vi "Drive Controller.vi"(8 "error in":errorcluster) -> ()   [LabVIEW 2023]
doc: "This VI executes continuously carrying out the current operation and responding to updates or new operation requests. It will often contain the timing or control code that is difficult to place directly in TeleOp. This VI generally opens all sensors and motors and isolates the rest of the robot code from knowing implementation details of how the operations are carried out."
uses:
  Drive Operations.ctl
  Drive Setpoints.ctl
  swerve-template/Type Definitions/Data/Robot Velocities.ctl
  Robot Global Data.vi
  80b923c8-6b82-42f9-a8cd-acddf0fa8107.vi
  Auto Data.ctl
  <vilib>/REV Custom Controls/Spark Output Control Type.ctl
  <vilib>/REVLibDriver/REVLibDriver.lvlib
panel:
  in  "Drive Controller Diagnostics":T1(tab)
  out "Swerve Visualizer":cluster{dbl[], dbl[]}[](graph)
  out "Pod Comparisons (Diff -> Setpoint - Actual)":T2
  out "(Calibration) Steering Angles":T3
  out "Current\nCmd":string
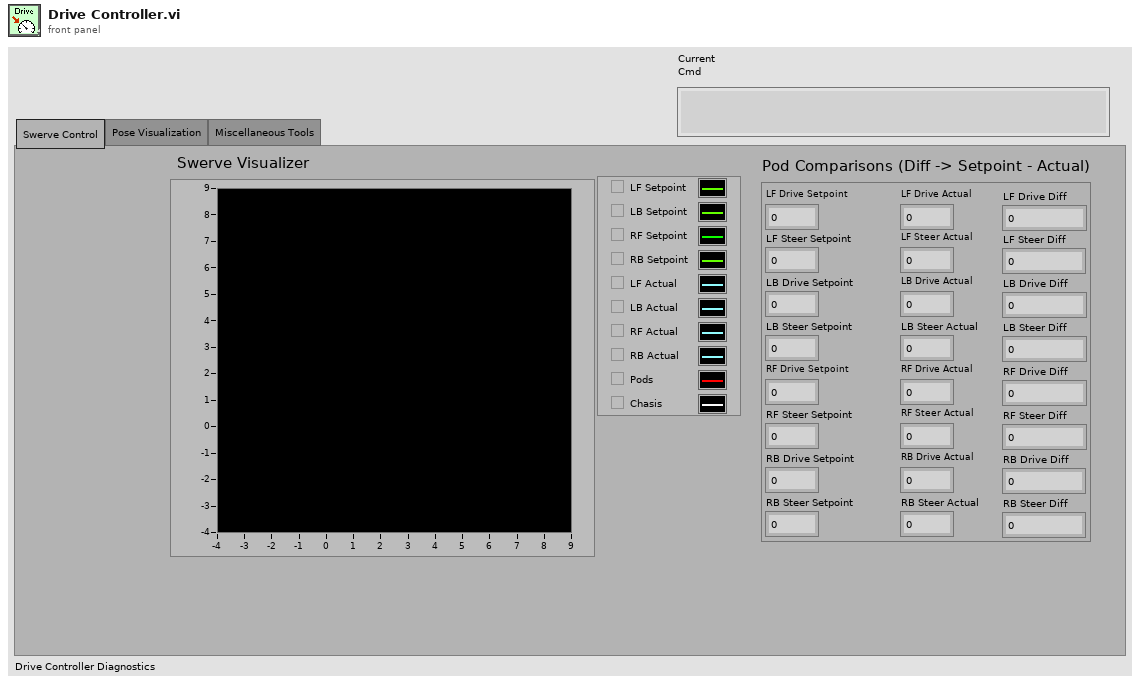
[diagram p1: front panel]
types:
  T1 = enum32{"Swerve Control", "Pose Visualization", "Miscellaneous Tools"}
  T2 = cluster{"LF Drive Setpoint":dbl, "LF Steer Setpoint":dbl, "LB Drive Setpoint":dbl, "LB Steer Setpoint":dbl, "RF Drive Setpoint":dbl, "RF Steer Setpoint":dbl, "RB Drive Setpoint":dbl, "RB Steer Setpoint":dbl, "LF Drive Actual":dbl, "LF Steer Actual":dbl, "LB Drive Actual":dbl, "LB Steer Actual":dbl, "RF Drive Actual":dbl, "RF Steer Actual":dbl, "RB Drive Actual":dbl, "RB Steer Actual":dbl, "LF Drive Diff":dbl, "LF Steer Diff":dbl, "LB Drive Diff":dbl, "LB Steer Diff":dbl, "RF Drive Diff":dbl, "RF Steer Diff":dbl, "RB Drive Diff":dbl, "RB Steer Diff":dbl}
  T3 = cluster{"Left Front":dbl, "Left Back":dbl, "Right Front":dbl, "Right Back":dbl}
  T4 = typedef "Drive Setpoints.ctl" = cluster{"Operation":T5, "Robot Velocities":T6, "Auto Data":T7}
  T5 = typedef "Drive Operations.ctl" = enum16{"Reserve", "Read Current", "Immediate", "Calibrate", "Auto", "Auto Pickup"}
  T6 = typedef "Robot Velocities.ctl" = cluster{"X Velocity":dbl, "Y Velocity":dbl, "Rotational \nVelocity":dbl}
  T7 = typedef "Auto Data.ctl" = cluster{"Auto Data":cluster{"Velocities":T6[], "Positions":cluster{"x":dbl, "y":dbl, "th":dbl}[], "Command Info":cluster{dbl, "Command out":cluster{"Name":string, "vi reference":refnum<vi>, i32[], variant[]}}[], "Zero Velocity?":bool[], "Zero Translational Velocity?":bool[], "Current Limit":dbl, "Correct at Beginning of Path":bool, "Name of Path":string}[], "Number of Remaining Auto Paths":dbl}
  T8 = typedef "(NEO-NEO-ThroughBore-Pigeon2) Swerve.ctl" = cluster{"Drive Motor IDs":cluster{"[0]":T9, "[1]":T9, "[2]":T9, "[3]":T9}, "Steer Motor IDs":cluster{"[0]":T9, "[1]":T9, "[2]":T9, "[3]":T9}, "Pod Locations (ft)":T10, "Drive Scaling":dbl, "Steer Scaling":dbl}
  T9 = typedef "REVLibDriver.lvlib/REVSparkRefnum.ctl" = refnum<k20>
  T10 = typedef "Pod Positions.ctl" = cluster{"Left Front Position":dbl[], "Left Back Position":dbl[], "Right Front Position":dbl[], "Right Back Position":dbl[]}
  T11 = typedef "Command Status Info.ctl" = cluster{"Name":string, "Status":T12, "notifier out":T13}
  T12 = typedef "Completion Status.ctl" = enum16{"Successful", "Aborted", "Incomplete"}
  T13 = typedef "Completion Notifier.ctl" = refnum<notifier>
  T14 = cluster{"SubSystem Data":T4, cluster{"Start Time (ms)":u32, "Iterations":i32}, cluster{"Command Info":T11, "Description":string, "Default Command":T4, "queue out":refnum<queue>, "Subsystem Name":string}}
  T15 = typedef "REVLibDriver.lvlib/Spark Output Control Type.ctl" = enum16{"Percent VBus", "Velocity", "Voltage", "Position", "Current", "MAXMotion Position", "MAXMotion Velocity"}
  T16 = cluster{"SubSystem Data":T4, cluster{"Start Time (ms)":u32, "Iterations":i32}, "Default Command Arguments":cluster{"Command Info":T11, "Description":string, "Default Command":T4, "queue out":refnum<queue>, "Subsystem Name":string}}
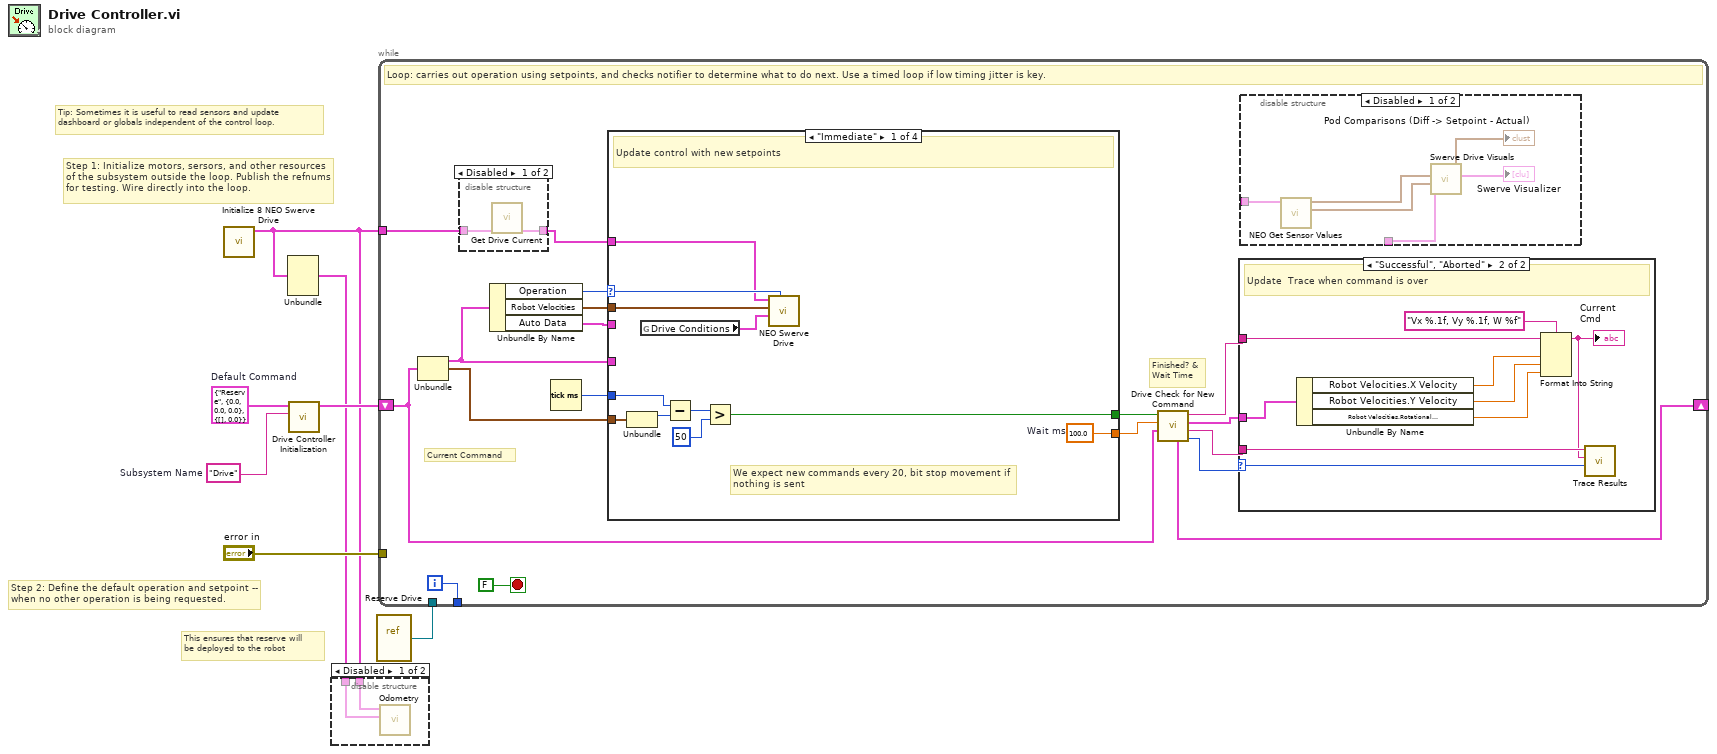
[diagram p0: block diagram]
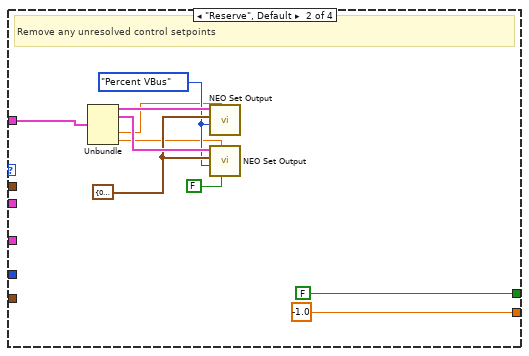
[diagram p4: hidden frame]
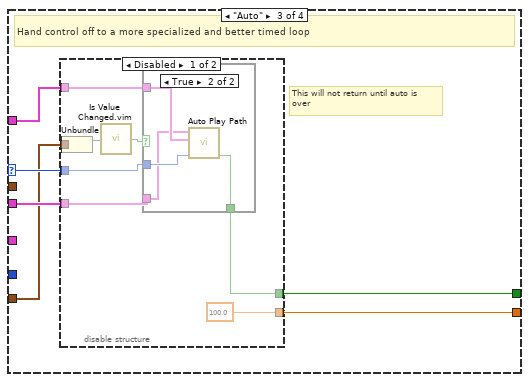
[diagram p5: hidden frame]
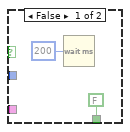
[diagram p6: hidden frame]
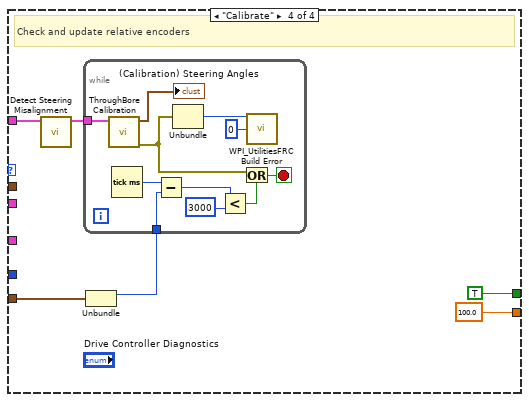
[diagram p8: hidden frame]
diagram:
  w3 = T4 {"Operation"=enum."Reserve", "Robot Velocities"={"X Velocity"=0.0, "Y Velocity"=0.0, "Rotational \nVelocity"=0.0}, "Auto Data"={"Auto Data"=[], "Number of Remaining Auto Paths"=0.0}}  # Default Command
  w7 = "Drive"  # Subsystem Name
  # "This ensures that reserve will\nbe deployed to the robot"
  # "Step 2: Define the default operation and setpoint --\nwhen no other operation is being requested."
  # "Step 1: Initialize motors, sersors, and other resources\nof the subsystem outside the loop. Publish the refnums\nfor testing. Wire directly into the loop."
  # "Tip: Sometimes it is useful to read sensors and update\ndashboard or globals independent of the control loop."
  n1 = call "Initialize 8 NEO Swerve Drive.vi"() -> ("(N-N-C-P) Swerve Motors"=w2:T8)  [unwired: 10 in, 1 out]
  n2 = Unbundle(w2) -> ("Pod Locations (ft)"=w1:T10)  [unwired: 4 out]
  n3 = call "Drive Controller Initialization.vi"("Subsystem Name"=w7, "Default Command"=w3) -> ("Current Command"=w5:T14)  [unwired: 9 in]
  n4 = disable-structure shown="Disabled" {
    disable-tunnel: w1 -> [w9 _]
    disable-tunnel: w2 -> [w8 _]
    frame Disabled {
      n5 = call "Odometry.vi"("Radii (ft)"=w9, "(N-N-C-P) Swerve Motors"=w8) -> ()  [unwired: 10 in]
    }
    frame Enabled {
    }
  }
  n6 = vi-ref "Reserve Drive.vi"() -> (w4:refnum<vi>)
  n7 = while {
    shift-right: [w20] -> _
    shift-left: w5 -> [w12]
    tunnel: [w26] -> _
    tunnel: "error in" -> [_]
    tunnel: w4 -> [_]
    tunnel: w2 -> [w11]
    i -> [w26]
    stop <- FALSE stop-if-true
    # "Current Command"
    # "Finished? &\nWait Time"
    # "Loop: carries out operation using setpoints, and checks notifier to determine what to do next. Use a timed loop if low timing jitter is key."
    n8 = Unbundle(w12) -> ("SubSystem Data"=w15:T4, w13:cluster{"Start Time (ms)":u32, "Iterations":i32})  [unwired: 1 out]
    n9 = disable-structure shown="Disabled" {
      disable-tunnel: w11 -> [w29 w30]
      disable-tunnel: [w28 w30] -> w10
      frame Disabled {
        n10 = call "Get Drive Current.vi"("Motors In"=w29) -> ("Motors Out"=w28:T8)  [unwired: 10 in]
      }
      frame Enabled {
      }
    }
    n11 = Unbundle By Name(w15) -> ("Operation"=w18:T5, "Robot Velocities"=w21:T6, "Auto Data"=w19:T7)
    n12 = Tick Count (ms)() -> (millisecond timer value=w14:u32)
    n13 = case shown="\"Immediate\"" w18 {
      selector: w18 -> [w33 _ w55 _]
      tunnel: [w41 -1.0 ("Infinite") w56 100.0 ("Infinite")] -> w25
      tunnel: [w36 FALSE ("ignore previous (F)") w54 TRUE ("ignore previous (F)")] -> w24
      tunnel: w13 -> [w40 _ w52 w75]
      tunnel: w14 -> [w35 _ _ _]
      tunnel: w21 -> [w32 _ _ _]
      tunnel: w10 -> [w31 w49 w57 w73]
      tunnel: w15 -> [_ _ _ _]
      tunnel: w19 -> [_ _ w53 _]
      frame "Immediate" {
        w41 = 100.0  # Wait ms
        # "We expect new commands every 20, bit stop movement if\nnothing is sent"
        # "Update control with new setpoints"
        n14 = Unbundle(w40) -> ("Start Time (ms)"=w39:u32)  [unwired: 1 out]
        n15 = global read "Robot Global Data.vi" "Drive Conditions"() -> (w34:cluster{"Field Centric":bool, "Reset PIDs":bool})
        n16 = Subtract(x=w35, y=w39) -> (x-y=w38:u32)
        n17 = Greater?(x=w38, y=u32 50) -> (0:w36:bool)
        n18 = call "NEO Swerve Drive.vi"("Operation"=w33, "Drive Conditions"=w34, "Robot Velocities"=w32, "Motors In"=w31) -> ()  [unwired: 6 in, 2 out]
      }
      frame "Reserve", Default {
        w44 = Spark_Output_Control_Type."Percent VBus" ("Control Mode")
        w45 = T3 {"Left Front"=0.0, "Left Back"=0.0, "Right Front"=0.0, "Right Back"=0.0} ("Setpoints")
        # "Remove any unresolved control setpoints"
        n19 = Unbundle(w49) -> ("Drive Motor IDs"=w48:cluster{"[0]":T9, "[1]":T9, "[2]":T9, "[3]":T9}, "Steer Motor IDs"=w47:cluster{"[0]":T9, "[1]":T9, "[2]":T9, "[3]":T9}, "Drive Scaling"=w43:dbl, "Steer Scaling"=w42:dbl)  [unwired: 1 out]
        n20 = call "NEO Set Output.vi"("Scaling"=w43, "Control Mode"=w44, "Setpoints"=w45, "Motors"=w48) -> ()  [unwired: 7 in, 1 out]
        n21 = call "NEO Set Output.vi"("Add Angle Offsets?"=FALSE, "Scaling"=w42, "Control Mode"=w44, "Setpoints"=w45, "Motors"=w47) -> ()  [unwired: 6 in, 1 out]
      }
      frame "Auto" {
        # "This will not return until auto is\nover"
        # "Hand control off to a more specialized and better timed loop"
        n22 = disable-structure shown="Disabled" {
          disable-tunnel: w57 -> [w65 _]
          disable-tunnel: [100.0 _] -> w56
          disable-tunnel: w55 -> [w61 _]
          disable-tunnel: [w60 _] -> w54
          disable-tunnel: w53 -> [w59 _]
          disable-tunnel: w52 -> [w58 _]
          frame Disabled {
            n23 = Unbundle(w58) -> ("Start Time (ms)"=w63:u32)  [unwired: 1 out]
            n24 = call "Is Value Changed.vim"("value"=w63) -> ("changed or first call?"=w62:bool)
            n25 = case shown="True" w62 {
              tunnel: w59 -> [_ w68]
              tunnel: w65 -> [_ w71]
              tunnel: w61 -> [_ w70]
              tunnel: [FALSE ("Auto Done?") w69] -> w60
              frame False {
                n26 = Wait (ms)(milliseconds to wait=u32 200) -> ()  [unwired: 1 out]
              }
              frame True {
                n27 = call "Auto Play Path.vi"("Operation"=w70, "(N-N-C-P) Swerve Motors"=w71, "Auto Data"=w68) -> ("Auto Done?"=w69:bool)  [unwired: 6 in, 2 out]
              }
            }
          }
          frame Enabled {
          }
        }
      }
      frame "Calibrate" {
        # "Check and update relative encoders"
        n28 = call "Detect Steering Misalignment.vi"("Motors In"=w73) -> ("Motors out"=w72:T8)  [unwired: 10 in]
        n29 = Unbundle(w75) -> ("Start Time (ms)"=w74:u32)  [unwired: 1 out]
        n30 = while {
          tunnel: w72 -> [w82]
          tunnel: w74 -> [w87]
          stop <- w88 stop-if-true
          n31 = call "ThroughBore Calibration.vi"("(N-N-C-P) Swerve Motors"=w82) -> ("error out"=w79:errorcluster, "Steering Angles"=→"(Calibration) Steering Angles":cluster{"LF":dbl, "LB":dbl, "RF":dbl, "RB":dbl})  [unwired: 9 in]
          n32 = Tick Count (ms)() -> (millisecond timer value=w86:u32)
          n33 = Subtract(x=w86, y=w87) -> (x-y=w85:u32)
          n34 = Unbundle(w79) -> ("code"=w78:i32)  [unwired: 2 out]
          n35 = Less?(x=w85, y=u32 3000) -> (x < y?=w83:bool)
          n36 = Or(x=w79, y=w83) -> (x .or. y?=w88:bool)
          n37 = call <vilib>:"WPI_UtilitiesFRC Build Error.vi"("error code"=w78, "chain levels to remove (1)"=0) -> ()  [unwired: 3 in, 11 out]
        }
      }
    }
    n38 = call "Drive Check for New Command.vi"("input cluster"=w12, "Wait time (ms)"=w25, "Finished?"=w24) -> ("Completion"=w17:T12, "Subsystem Name"=w22:string, "Current Command"=w16:T4, "Initial Trace String"=w23:string, "Next Command"=w20:T16)  [unwired: 4 in]
    n39 = case shown="\"Successful\", \"Aborted\"" w17 {
      selector: w17 -> [_ w95]
      tunnel: w23 -> [_ w102]
      tunnel: w16 -> [_ w103]
      tunnel: w22 -> [_ w101]
      frame "Incomplete", Default {
        # "Continuing current command"
      }
      frame "Successful", "Aborted" {
        # "Update  Trace when command is over"
        n40 = Unbundle By Name(w103) -> ("Robot Velocities.X Velocity"=w99:dbl, "Robot Velocities.Y Velocity"=w100:dbl, "Robot Velocities.Rotational \nVelocity"=w96:dbl)
        n41 = Format Into String(format string="Vx %.1f, Vy %.1f, W %f", initial string=w102, w99, w100, w96) -> (resulting string=w97:string)  [unwired: 1 in, 1 out]
        "Current\nCmd" <- w97
        n42 = call <vilib>:"Trace Results.vi"("Status of previous command"=w95, "Description"=w97, "Subsystem"=w101) -> ()  [unwired: 9 in]
      }
    }
    n43 = disable-structure shown="Disabled" {
      disable-tunnel: _ -> [w92 _]
      disable-tunnel: _ -> [w89 _]
      frame Disabled {
        n44 = call "NEO Get Sensor Values.vi"("Motors In"=w89) -> ("Steer Angles (degrees)"=w90:T3, "Drive Velocities (ft/s)"=w91:T3)  [unwired: 9 in]
        n45 = call "Swerve Drive Visuals.vi"("Steer Angles (degrees)"=w90, "Drive Velocities (ft/s)"=w91, "Pod Setpoints (ft/s and deg)"=w92) -> ("Swerve Visualizer"=→"Swerve Visualizer":cluster{dbl[], dbl[]}[], "Pod Comparisons (Diff -> Setpoint - Actual)"=→"Pod Comparisons (Diff -> Setpoint - Actual)":T2)  [unwired: 7 in]
      }
      frame Enabled {
      }
    }
  }
